vi "Destroy.vi"(0 "ClassWriterGOOP300.lvclass":refnum<class "ClassWriterGOOP300.lvclass">, 5 "error in (no error)":errorcluster) -> (19 "error out":errorcluster)   [LabVIEW 2020, in "ClassWriterGOOP300.lvclass"]
doc: "Destroys a ClassWriterNative object created with a ClassWriterNative constructor VI.\n\n[GOOP 2.0.16]"
uses:
  ClassWriterGOOP300.lvclass
  Provider_LvNativeClass/ClassWriterNative_class/ClassWriterNative.lvclass
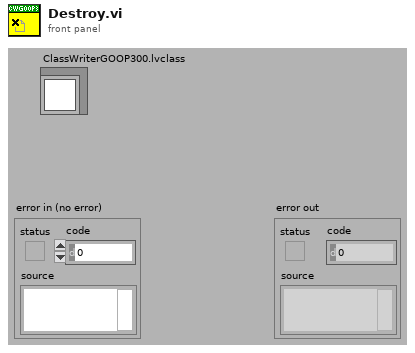
[diagram p1: front panel]
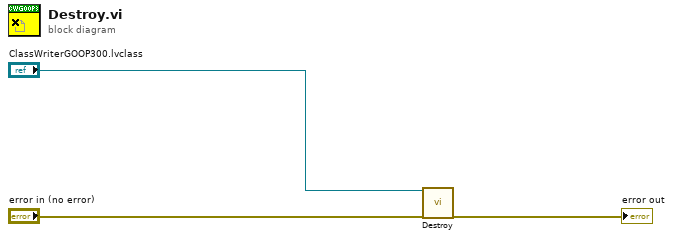
[diagram p0: block diagram]
diagram:
  n1 = call-parent "Destroy.vi"("ClassWriterNative"="ClassWriterGOOP300.lvclass", "error in (no error)"="error in (no error)") -> ("error out"=→"error out":errorcluster)  [unwired: 17 in]
